vi "Compare File with Master.vi"(8 "error in":errorcluster, 10 "File Index":i32, 11 "Peer Review in":refnum<class "Peer Review.lvclass">) -> (0 "error out":errorcluster, 3 "Peer Review out":refnum<class "Peer Review.lvclass">)   [LabVIEW 2020, in "Peer Review.lvclass"]
uses:
  Peer Review.lvclass
  Peer Review.lvclass/Peer Review.ctl
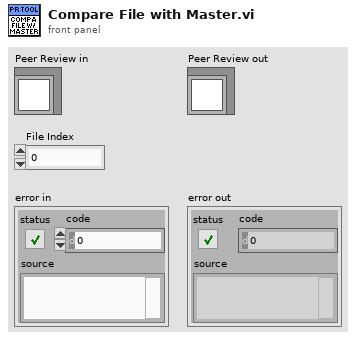
[diagram p1: front panel]
types:
  T1 = typedef "Peer Review.lvclass/File Info.ctl" = cluster{"File ID":i32, "Commit ID":i32, "Reviewed Hash":string, "Relative Path":string, "File Path":path, "File Checksum":string, "State":T2, "FP Changes":i32, "BD Changes":i32, "FP Bounds Error":dbl, "BD Bounds Error":dbl, "Lines Added":i32, "Lines Removed":i32, "Analysis Passes":i32, "Analysis Fails":i32, "Attribute Changes":i32, "Reentrancy State":string, "Cyclomatic Complexity":i32, "Node Count":i32, "Revision Number":u32, "LabVIEW Version":string, "Description":string, "Master Path":path, "Master Checksum":string, "VI Type":T3, "LabVIEW File":bool, "Review Complete":bool, "File Ref":refnum<vi>}
  T2 = typedef "Peer Review.lvclass/File State.ctl" = enum16{"Interrogation Needed", "Modified", "Deleted", "Added", "Matches Previous", "No Changes", "Moved"}
  T3 = typedef "Peer Review.lvclass/VI Type.ctl" = enum32{"invalid VI type", "Standard VI", "Control VI", "Global VI", "Polymorphic VI", "Configuration VI", "SubSystem", "Facade VI", "Method VI", "Statechart Diagram VI"}
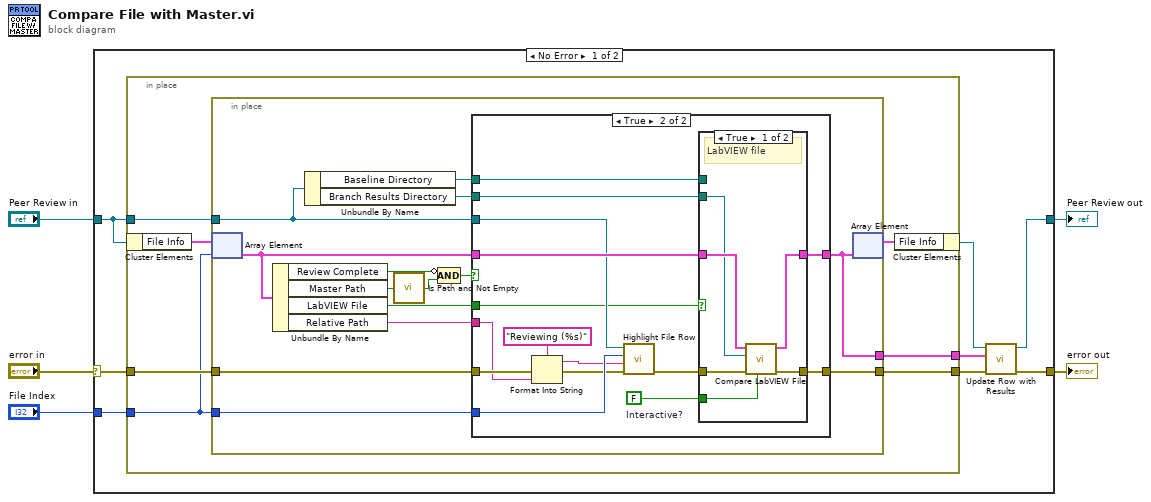
[diagram p0: block diagram]
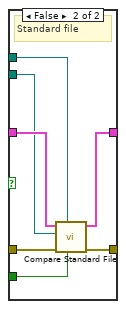
[diagram p3: hidden frame]
diagram:
  n1 = case shown="No Error" "error in" {
    selector: "error in" -> [w11 w66]
    tunnel: [w12 w66] -> w4
    tunnel: "Peer Review in" -> [w8 w65]
    tunnel: "File Index" -> [w13 _]
    tunnel: [w6 w65] -> w1
    frame No Error {
      n2 = in-place {
        in-place-border: w13 -> [w15]
        in-place-border: w11 -> [w20]
        in-place-border: w8 -> [w19]
        in-place-border: [w18] -> w10
        in-place-border: [w17] -> w9
        n3 = in-place-cluster #1(w8) -> ("File Info"=w16:T1[])
        n4 = in-place {
          in-place-border: w15 -> [w32]
          in-place-border: w20 -> [w34]
          in-place-border: w19 -> [w23]
          in-place-border: [w33] -> w18
          in-place-border: [w31] -> w17
          n5 = in-place-array #2(w16, w15) -> (w30:T1)
          n6 = Unbundle By Name(w30) -> ("Review Complete"=w29:bool, "Master Path"=w27:path, "LabVIEW File"=w25:bool, "Relative Path"=w24:string)
          n7 = Unbundle By Name(w23) -> ("Baseline Directory"=w22:path, "Branch Results Directory"=w21:path)
          n8 = call <vilib>:"Is Path and Not Empty.vi"("path"=w27) -> ("Is Path and Not Empty?"=w26:bool)  [unwired: 4 in]
          n9 = Compound Arithmetic op=AND(invert w29, w26) -> (w28:bool)
          n10 = case shown="True" w28 {
            tunnel: w34 -> [w35 w51]
            tunnel: [w35 w50] -> w33
            tunnel: [w36 w49] -> w31
            tunnel: w23 -> [_ w45]
            tunnel: w32 -> [_ w47]
            tunnel: w30 -> [w36 w46]
            tunnel: w25 -> [_ w40]
            tunnel: w24 -> [_ w39]
            tunnel: w22 -> [_ w38]
            tunnel: w21 -> [_ w37]
            frame False {
              # "Do nothing since this file has already been reviewed or no master to compare against."
            }
            frame True {
              w41 = FALSE  # Interactive?
              n11 = Format Into String(format string="Reviewing (%s)", error in=w51, w39) -> (resulting string=w44:string, error out=w43:errorcluster)  [unwired: 1 in]
              n12 = call "Highlight File Row.vi"("error in"=w43, "Status"=w44, "Current Row"=w47, "Peer Review"=w45) -> ("error out"=w48:errorcluster)  [unwired: 7 in]
              n13 = case shown="True" w40 {
                tunnel: w48 -> [w57 w64]
                tunnel: [w56 w63] -> w50
                tunnel: [w55 w62] -> w49
                tunnel: w41 -> [w52 w60]
                tunnel: w46 -> [w54 w61]
                tunnel: w37 -> [w53 w59]
                tunnel: w38 -> [_ w58]
                frame True {
                  # "LabVIEW file"
                  n14 = call "Compare LabVIEW File.vi"("Interactive?"=w52, "error in"=w57, "Results Directory"=w53, "File Info in"=w54) -> ("error out"=w56:errorcluster, "File Info out"=w55:T1)  [unwired: 6 in]
                }
                frame False {
                  # "Standard file"
                  n15 = call "Compare Standard File.vi"("Interactive?"=w60, "Baseline Directory"=w58, "error in"=w64, "Results Directory"=w59, "File Info in"=w61) -> ("error out"=w63:errorcluster, "File Info out"=w62:T1)  [unwired: 5 in]
                }
              }
            }
          }
          n16 = in-place-array #2(w31) -> (w14:T1[])  [unwired: 1 out]
        }
        n17 = in-place-cluster #1("File Info"=w14) -> (w7:refnum<class "Peer Review.lvclass">)
      }
      n18 = call "Update Row with Results.vi"("error in"=w10, "File Info"=w9, "Peer Review in"=w7) -> ("error out"=w12:errorcluster, "Peer Review out"=w6:refnum<class "Peer Review.lvclass">)  [unwired: 7 in]
    }
    frame Error {
    }
  }
  "error out" <- w4
  "Peer Review out" <- w1
